vi "Add Tag.vi"(8 "error in (no error)":errorcluster, 10 "Tag in":refnum<class "Tag.lvclass">) -> (0 "error out":errorcluster, 2 "Tag Reference out":refnum<data-value>)   [LabVIEW 2020, in "Tag Engine Core.lvlib" / "Tag Core.lvclass"]
doc: "_SubVI_"
uses:
  Tag Core.lvclass
  Tag/Tag.lvclass
  Tag Core.lvclass/Tag Core.ctl
  Tag/Tag.lvclass/Tag.ctl
  Tag/Read Name.vi
  <vilib>/Utility/error.llb/Error Cluster From Error Code.vi
  <vilib>/ErrorRing/Error Ring.xnode
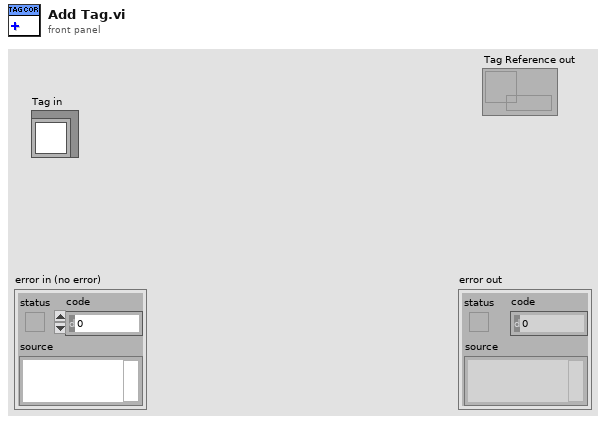
[diagram p1: front panel]
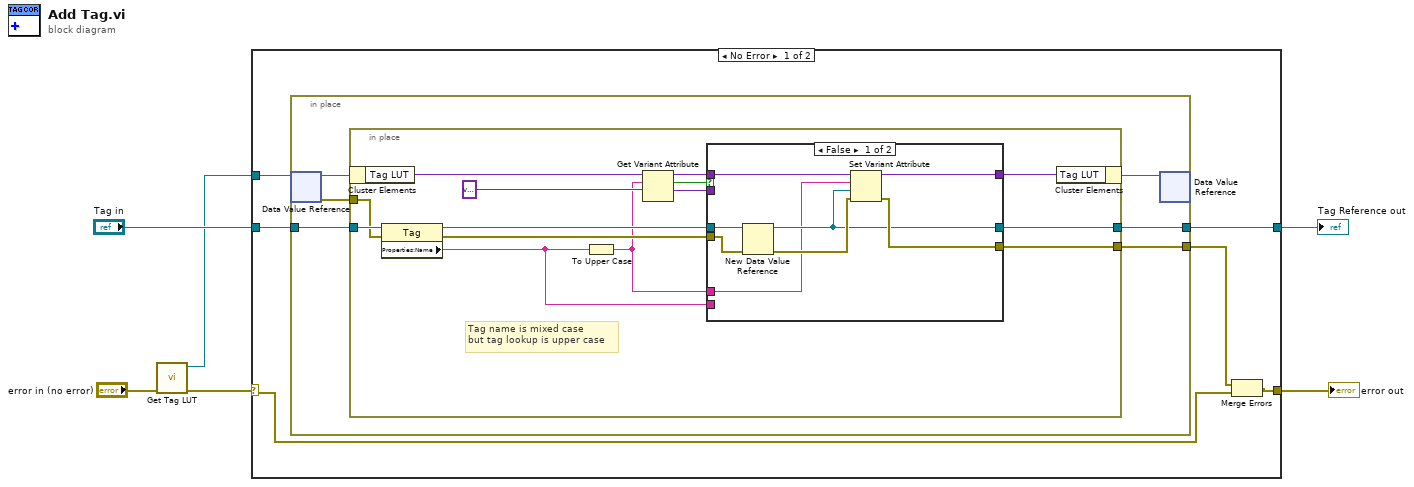
[diagram p0: block diagram]
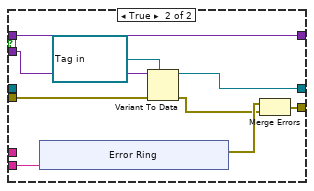
[diagram p2: hidden frame]
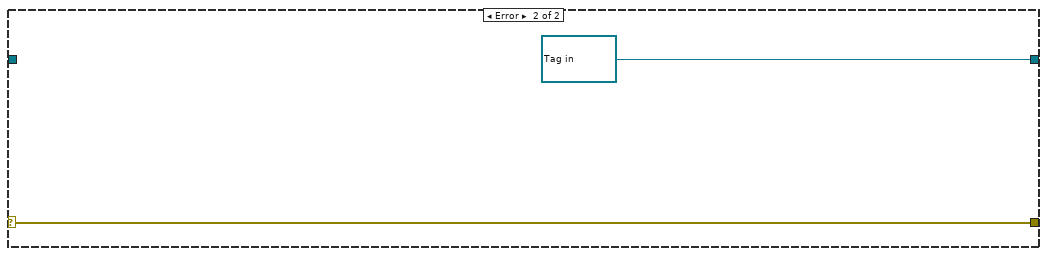
[diagram p3: hidden frame]
diagram:
  n1 = call "Get Tag LUT.vi"("error in (no error)"="error in (no error)") -> ("error out"=w5:errorcluster, "Tag LUT Out"=w3:refnum<data-value>)  [unwired: 9 in]
  n2 = case shown="No Error" w5 {
    selector: w5 -> [w9 w57]
    tunnel: "Tag in" -> [w11 _]
    tunnel: w3 -> [w12 _]
    tunnel: [w8 w57] -> w2
    tunnel: [w7 refnum<data-value> refnum ("data value reference")] -> w1
    frame No Error {
      n3 = in-place {
        in-place-border: w11 -> [w17]
        in-place-border: [w15] -> w10
        in-place-border: [w13] -> w7
        n4 = in-place-dvr #1(w12) -> (w18:refnum<class "Tag Core.lvclass">, w14:errorcluster)
        n5 = in-place {
          in-place-border: w17 -> [w32]
          in-place-border: [w27] -> w15
          in-place-border: w14 -> [w26]
          in-place-border: [w25] -> w13
          # "Tag name is mixed case\nbut tag lookup is upper case"
          n6 = in-place-cluster #2(w18) -> ("Tag LUT"=w31:variant)
          n7 = property class="Tag"(reference=w32, error in=w26) -> (reference out=w22:refnum<class "Tag.lvclass">, error out=w21:errorcluster, "Properties:Name"=w19:string)
          n8 = To Upper Case(1:w19) -> (0:w20:string)
          n9 = Get Variant Attribute(Variant=w31, name=w20, default value (empty Variant)=variant ("default value (empty variant)")) -> (duplicate Variant=w29:variant, found=w30:bool, value=w23:variant)  [unwired: 1 in, 1 out]
          n10 = case shown="False" w30 {
            tunnel: w29 -> [w39 w48]
            tunnel: w22 -> [w40 _]
            tunnel: w21 -> [w38 w46]
            tunnel: w20 -> [w33 _]
            tunnel: [w36 w48] -> w28
            tunnel: [w35 w47] -> w27
            tunnel: [w34 w43] -> w25
            tunnel: w23 -> [_ w44]
            tunnel: w19 -> [_ w41]
            frame False {
              n11 = New Data Value Reference(data value=w40, error in=w38) -> (data value reference=w34:refnum<data-value>, error out=w37:errorcluster)
              n12 = Set Variant Attribute(Variant=w39, name=w33, value=w34, error in=w37) -> (Variant out=w36:variant, error out=w35:errorcluster)  [unwired: 1 out]
            }
            frame True {
              n13 = xnode "Error Ring"("parameter 0"=w41) -> ("error out"=w49:errorcluster)
              n14 = Variant To Data(error in=w46, type=refnum<data-value> refnum ("data value reference"), Variant=w44) -> (data=w43:refnum<data-value>, error out=w45:errorcluster)
              n15 = Merge Errors(w49, w45) -> (w47:errorcluster)
            }
          }
          n16 = in-place-cluster #2("Tag LUT"=w28) -> (w16:refnum<class "Tag Core.lvclass">)
        }
        n17 = in-place-dvr #1(w16) -> ()  [unwired: 2 out]
      }
      n18 = Merge Errors(w10, w9) -> (w8:errorcluster)
    }
    frame Error {
    }
  }
  "error out" <- w2
  "Tag Reference out" <- w1
